vi "TagExpr_general.utest.vi"() -> ()   [LabVIEW 2020]
doc: "_Test_"
uses:
  Tag Expr/Tag Expr.lvclass
  C:/Program Files (x86)/National Instruments/LabVIEW 2020/vi.lib/LAVA/muParser/mupExpr/mupExpr.lvclass
  Tag/Tag.lvclass/Tag.ctl
  Tag Expr/Tag Expr.lvclass/Tag Expr.ctl
  <vilib>/LAVA/muParser/mupExpr/mupExpr.lvclass/mupExpr.ctl
  2f2ee43f-0975-4879-873a-ea0bf2c8b65a.vi
  ca224119-05c6-41cf-9db8-ad80aa452f58.vi
  Tag Expr/Read TagVarNames.vi
  <vilib>/LAVA/muParser/mupExpr/Eval.vi
  <vilib>/LAVA/muParser/mupExpr/Eval_SglRes.vi
  Tag Expr/Lookup Tag Values.vi
  Tag/Read Name.vi
  <vilib>/LAVA/muParser/mupLib/mupEval.vi
  API/Get Tag Value_ByRef.vi
  <vilib>/LAVA/muParser/mupExpr/Set_Var_Value.vi
  <vilib>/LAVA/muParser/mupExpr/Set_MultiVar_Value.vi
  <vilib>/LAVA/muParser/mupLib/mupCheckError.vi
  Tag/Read Value.vi
  Tag/Read Timestamp.vi
  <vilib>/LAVA/muParser/mupExpr/SetVarVal.vi
  <vilib>/LAVA/muParser/mupLib/mupSetVarValue.vi
  Core/Get Delimiter.vi
  <vilib>/Utility/error.llb/Error Cluster From Error Code.vi
  Tag/Set Properties from Initial.vi
  Core/Add Tag.vi
  <vilib>/addons/_JKI Toolkits/Caraya/classes/Assert/Assert Equal Value_Variant.vi
  <vilib>/addons/_JKI Toolkits/Caraya/classes/Assert/Assert Not Error.vi
  Tag/Tag.lvclass
  Tag Engine.lvlib
  <vilib>/addons/_JKI Toolkits/Caraya/classes/Test/Test.lvclass
  <vilib>/addons/_JKI Toolkits/Caraya/classes/Assert/Assert.lvclass
panel:
  out "Tag Names":string[](array[string])
  out "Expression readback":string
  out "Result":dbl format="%#_13g"
  out "error out":errorcluster
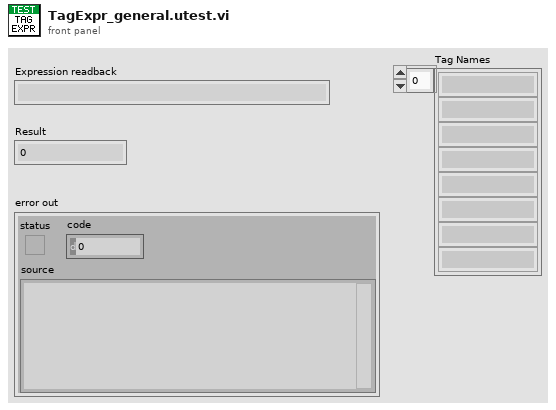
[diagram p1: front panel]
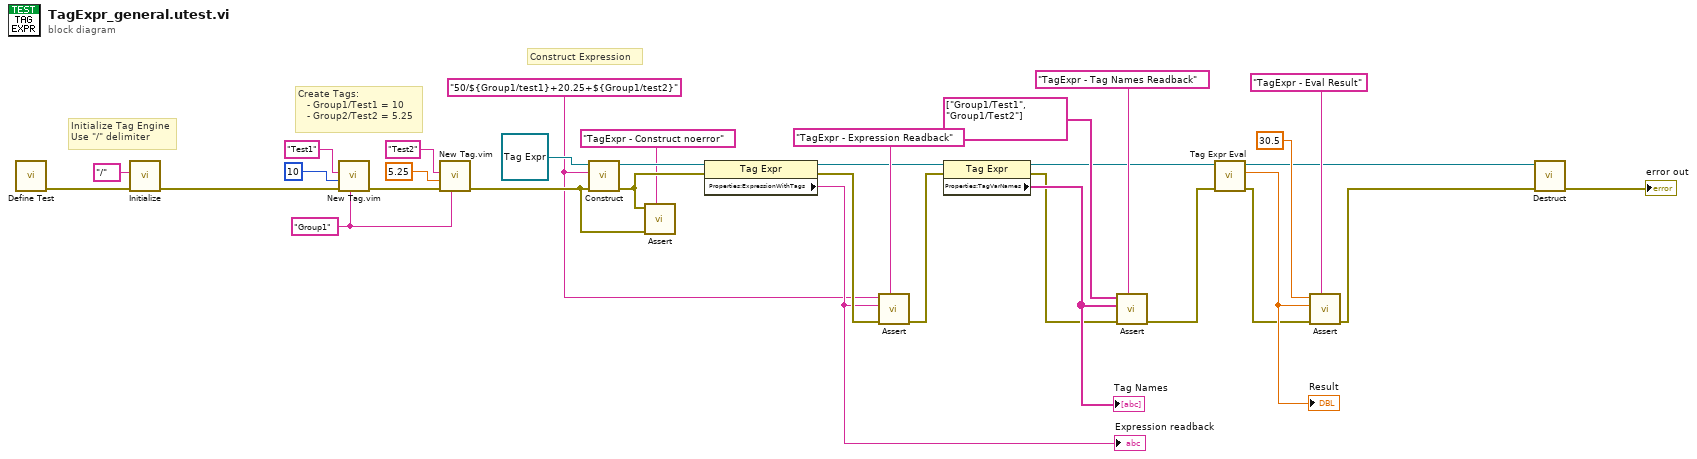
[diagram p0: block diagram]
diagram:
  w15 = "50/${Group1/test1}+20.25+${Group1/test2}" ("Expression")
  w24 = "Group1" ("Namespace")
  # "Construct Expression"
  # "Create Tags:\n   - Group1/Test1 = 10\n   - Group2/Test2 = 5.25"
  # "Initialize Tag Engine\nUse \"/\" delimiter"
  n1 = call <vilib>:"Define Test.vi"() -> ("error out"=w30:errorcluster)  [unwired: 10 in, 1 out]
  n2 = call "Initialize.vi"("error in (no error)"=w30, "Namespace Delimiter"="/") -> ("error out"=w32:errorcluster)  [unwired: 9 in]
  n3 = call "New Tag.vim"("Namespace"=w24, "error in (no error)"=w32, "Initial Value"=10, "Tag Name"="Test1" ("Name")) -> ("error out"=w25:errorcluster)  [unwired: 6 in, 1 out]
  n4 = call "New Tag.vim"("Namespace"=w24, "error in (no error)"=w25, "Initial Value"=5.25, "Tag Name"="Test2" ("Name")) -> ("error out"=w22:errorcluster)  [unwired: 6 in, 1 out]
  n5 = call-dynamic "Construct.vi"("error in (no error)"=w22, "Expression"=w15, "Tag Expr in"=refnum<class "Tag Expr.lvclass"> refnum ("CVT Engine:CVT Expr.lvclass")) -> ("error out"=w20:errorcluster, "Tag Expr out"=w21:refnum<class "Tag Expr.lvclass">)  [unwired: 5 in, 2 out]
  n6 = call-poly <vilib>:"Assert.vi"("Label"="TagExpr - Construct noerror", "error in (no error)"=w22, "Not Error?"=w20) -> ()  [unwired: 7 in, 2 out]
  n7 = property on="Property Node" class="Tag Expr"(reference=w21, error in=w20) -> (reference out=w12:refnum<class "Tag Expr.lvclass">, error out=w19:errorcluster, "Properties:ExpressionWithTags"=w16:string)
  "Expression readback" <- w16
  n8 = call-poly <vilib>:"Assert.vi"("Label"="TagExpr - Expression Readback", "error in (no error)"=w19, "Actual"=w16, "Expected"=w15) -> ("error out"=w11:errorcluster)  [unwired: 6 in, 1 out]
  n9 = property on="Property Node" class="Tag Expr"(reference=w12, error in=w11) -> (reference out=w8:refnum<class "Tag Expr.lvclass">, error out=w9:errorcluster, "Properties:TagVarNames"=w10:string[])
  "Tag Names" <- w10
  n10 = call-poly <vilib>:"Assert.vi"("Label"="TagExpr - Tag Names Readback", "error in (no error)"=w9, "Actual"=w10, "Expected"=string[] ["Group1/Test1", "Group1/Test2"]) -> ("error out"=w7:errorcluster)  [unwired: 6 in, 1 out]
  n11 = call "Tag Expr Eval.vi"("error in (no error)"=w7, "Tag Expr in"=w8) -> ("error out"=w5:errorcluster, "Result"=w6:dbl, "Tag Expr out"=w1:refnum<class "Tag Expr.lvclass">)  [unwired: 6 in, 1 out]
  "Result" <- w6
  n12 = call-poly <vilib>:"Assert.vi"("Label"="TagExpr - Eval Result", "error in (no error)"=w5, "Actual"=w6, "Expected"=30.5) -> ("error out"=w2:errorcluster)  [unwired: 6 in, 1 out]
  n13 = call-dynamic "Destruct.vi"("error in (no error)"=w2, "muExpr in"=w1) -> ("error out"=→"error out":errorcluster)  [unwired: 9 in]
